vi "onComputeIntervals.vi"(8 "error in (no error)":errorcluster, 9 "Cron Interval":T1, 10 "Expression":string, 11 "Cron.Quartz in":refnum<class "Cron.Quartz.lvclass">) -> (0 "error out":errorcluster, 2 "Interval Parameters":T2, 3 "Cron.Quartz out":refnum<class "Cron.Quartz.lvclass">)   [LabVIEW 2013, in "openCron.lvlib" / "Cron.Quartz.lvclass"]
uses:
  Cron.Quartz.lvclass
  Cron/Cron Interval -- cluster.ctl
  Cron/Cron Interval -- enum.ctl
  Cron/Cron.lvclass
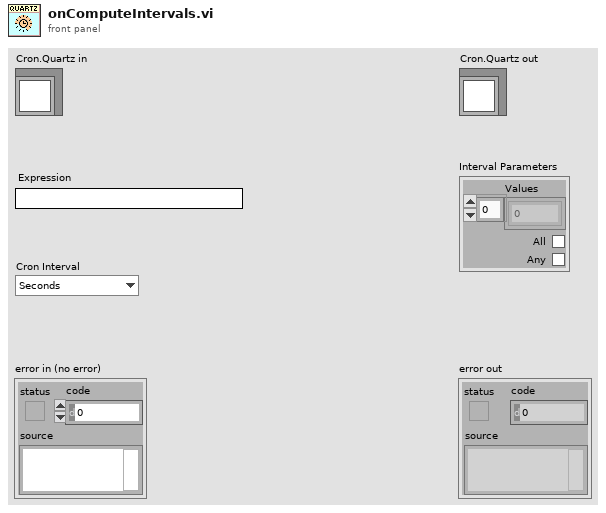
[diagram p1: front panel]
types:
  T1 = typedef "openCron.lvlib/Cron.lvclass/Cron Interval -- enum.ctl" = enum16{"Seconds", "Minutes", "Hours", "Day of Month", "Month", "Day of Week", "Year"}
  T2 = typedef "openCron.lvlib/Cron.lvclass/Cron Interval -- cluster.ctl" = cluster{"Values":i32[], "All":bool, "Any":bool}
  T3 = enum16{"SUN", "MON", "TUE", "WED", "THU", "FRI", "SAT"}
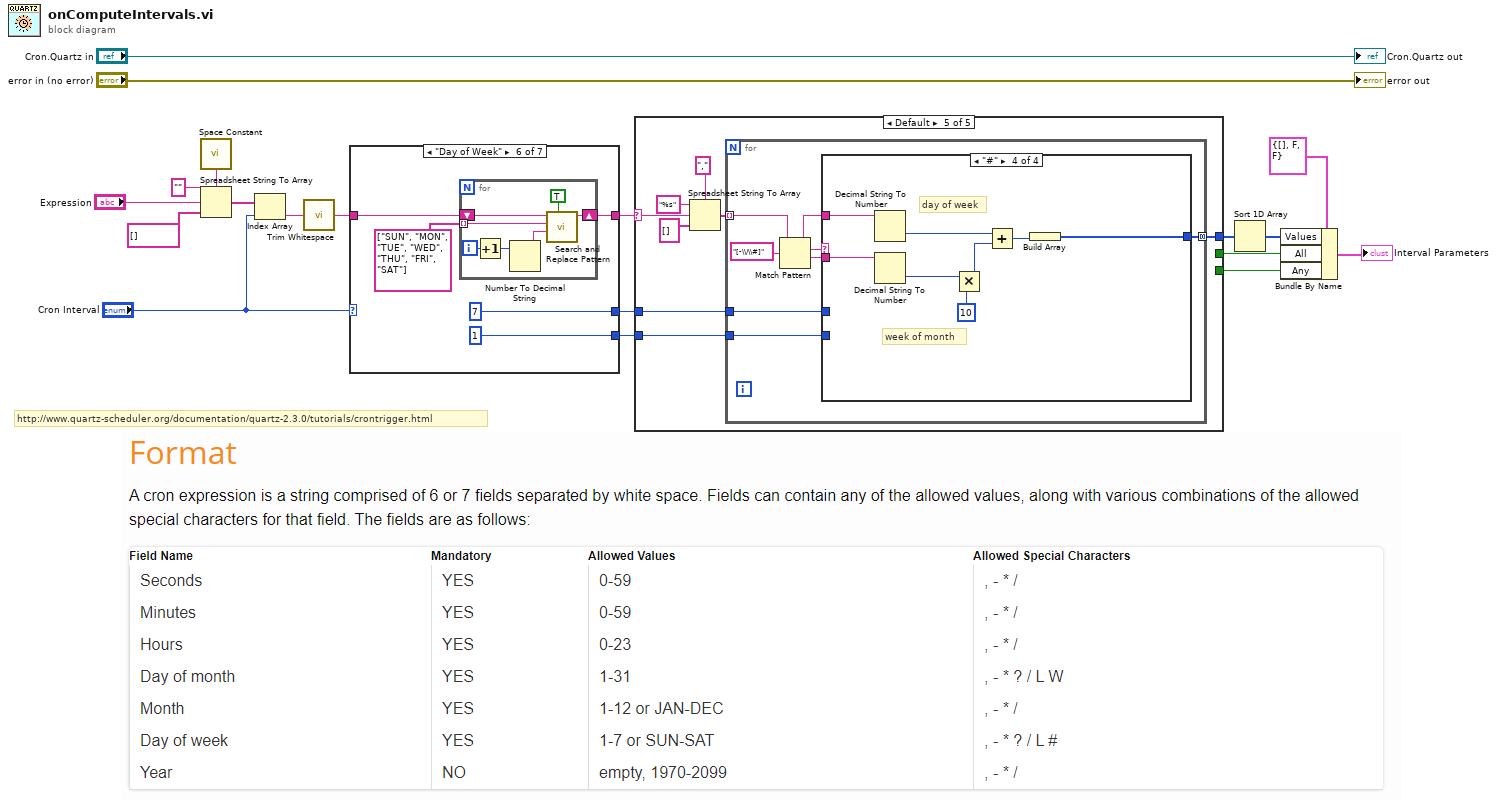
[diagram p0: block diagram]
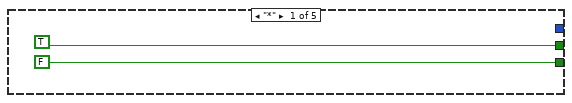
[diagram p2: hidden frame]
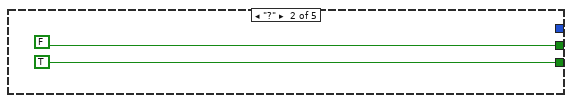
[diagram p3: hidden frame]
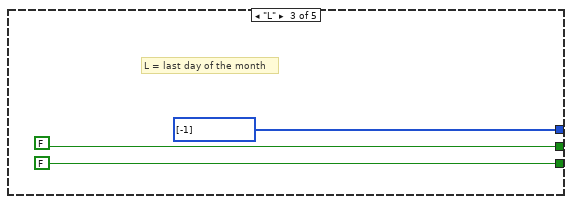
[diagram p4: hidden frame]
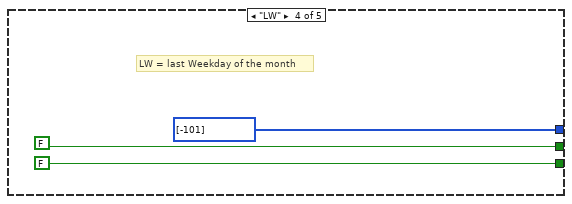
[diagram p5: hidden frame]
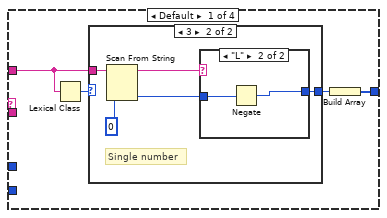
[diagram p6: hidden frame]
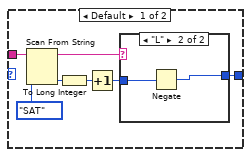
[diagram p7: hidden frame]
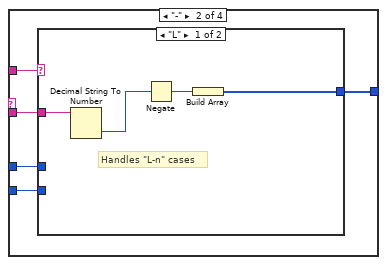
[diagram p10: hidden frame]
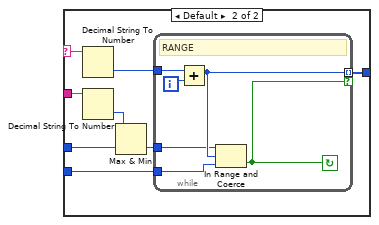
[diagram p11: hidden frame]
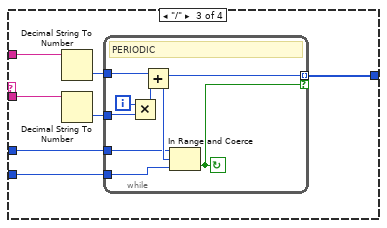
[diagram p12: hidden frame]
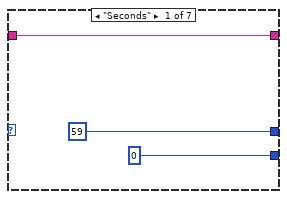
[diagram p13: hidden frame]
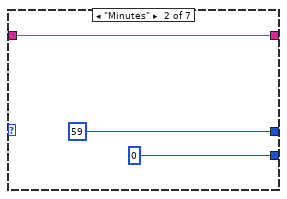
[diagram p14: hidden frame]
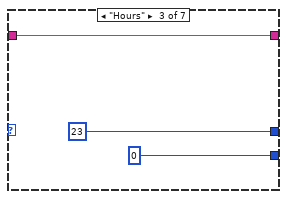
[diagram p15: hidden frame]
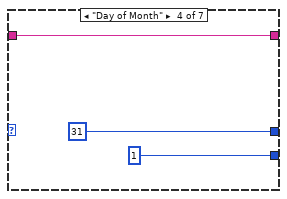
[diagram p16: hidden frame]
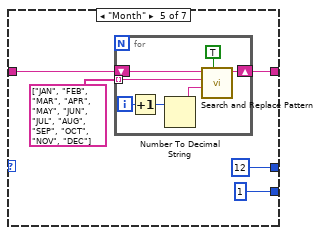
[diagram p17: hidden frame]
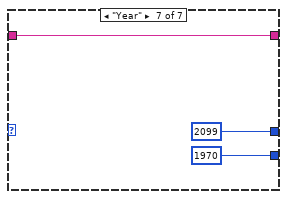
[diagram p18: hidden frame]
diagram:
  # "http://www.quartz-scheduler.org/documentation/quartz-2.3.0/tutorials/crontrigger.html"
  n1 = call <vilib>:"Space Constant.vi"() -> ("String"=w14:string)
  n2 = Spreadsheet String To Array(delimiter (Tab)=w14, format string="", spreadsheet string="Expression", array type (2D Dbl)=string[] []) -> (array=w13:string[])
  n3 = Index Array(array=w13, index="Cron Interval") -> (element=w11:string)
  n4 = call <vilib>:"Trim Whitespace.vi"("string"=w11) -> ("trimmed string"=w2:string)  [unwired: 1 in]
  n5 = case shown="\"Day of Week\"" "Cron Interval" {
    tunnel: [59 ("y") 59 ("y") 23 ("y") 31 ("y") 12 ("y") 7 ("y") 2099 ("y")] -> w10
    tunnel: [0 ("y") 0 ("y") 0 ("y") 1 ("y") 1 ("y") 1 ("y") 1970 ("y")] -> w9
    tunnel: w2 -> [w20 w23 w26 w29 w33 w45 w56]
    tunnel: [w20 w23 w26 w29 w34 w44 w56] -> w1
    frame "Seconds" {
    }
    frame "Minutes" {
    }
    frame "Hours" {
    }
    frame "Day of Month" {
    }
    frame "Month" {
      n6 = for {
        shift-right: [w43] -> w34
        shift-left: w33 -> [w42]
        tunnel: string[] ["JAN", "FEB", "MAR", "APR", "MAY", "JUN", "JUL", "AUG", "SEP", "OCT", "NOV", "DEC"] -> [w40] mode=indexing
        i -> [w39]
        n7 = Increment(x=w39) -> (x+1=w38:i32)
        n8 = Number To Decimal String(number=w38) -> (decimal integer string=w37:string)  [unwired: 1 in]
        n9 = call <vilib>:"Search and Replace Pattern.vi"("string"=w42, "regular expression (\"\")"=w40, "replace string (\"\")"=w37, "replace all? (F)"=TRUE) -> ("result string"=w43:string)  [unwired: 1 in, 1 out]
      }
    }
    frame "Day of Week" {
      n10 = for {
        shift-right: [w55] -> w44
        shift-left: w45 -> [w54]
        tunnel: string[] ["SUN", "MON", "TUE", "WED", "THU", "FRI", "SAT"] -> [w52] mode=indexing
        i -> [w51]
        n11 = Increment(x=w51) -> (x+1=w50:i32)
        n12 = Number To Decimal String(number=w50) -> (decimal integer string=w49:string)  [unwired: 1 in]
        n13 = call <vilib>:"Search and Replace Pattern.vi"("string"=w54, "regular expression (\"\")"=w52, "replace string (\"\")"=w49, "replace all? (F)"=TRUE) -> ("result string"=w55:string)  [unwired: 1 in, 1 out]
      }
    }
    frame "Year" {
    }
  }
  n14 = case shown="Default" w1 {
    selector: w1 -> [_ _ _ _ w72]
    tunnel: [_ _ i32[] [-1] i32[] [-101] w71] -> w7
    tunnel: [TRUE FALSE FALSE FALSE _] -> w6
    tunnel: [FALSE TRUE FALSE FALSE _] -> w5
    tunnel: w10 -> [_ _ _ _ w70]
    tunnel: w9 -> [_ _ _ _ w69]
    frame "*" {
    }
    frame "?" {
    }
    frame "L" {
      # "L = last day of the month"
    }
    frame "LW" {
      # "LW = last Weekday of the month"
    }
    frame Default {
      n15 = Spreadsheet String To Array(delimiter (Tab)=",", format string="%s", spreadsheet string=w72, array type (2D Dbl)=string[] []) -> (array=w73:string[])
      n16 = for {
        tunnel: w73 -> [w84] mode=indexing
        tunnel: [w80] -> w71 mode=concatenating
        tunnel: w70 -> [w78]
        tunnel: w69 -> [w77]
        n17 = Match Pattern(string=w84, regular expression="[-\\/\\#]") -> (before substring=w81:string, match substring=w82:string, after substring=w79:string)  [unwired: 1 in, 1 out]
        n18 = case shown="\"#\"" w82 {
          tunnel: w81 -> [w86 w107 w136 w152]
          tunnel: [w87 w110 w134 w150] -> w80
          tunnel: w79 -> [_ w111 w132 w151]
          tunnel: w78 -> [_ w109 w131 _]
          tunnel: w77 -> [_ w108 w130 _]
          frame Default {
            n19 = Lexical Class(1:w86) -> (0:w85:i16)
            n20 = case shown="3" w85 {
              tunnel: [w89 w101] -> w88
              tunnel: w86 -> [w95 w103]
              frame Default {
                n21 = Scan From String(input string=w95, default 1=T3."SAT" ("y")) -> (remaining string=w91:string, output 1=w92:T3)  [unwired: 3 in, 2 out]
                n22 = To Long Integer(number=w92) -> (32bit integer=w93:i32)
                n23 = Increment(x=w93) -> (x+1=w90:i32)
                n24 = case shown="\"L\"" w91 {
                  tunnel: w90 -> [w96 w98]
                  tunnel: [w96 w97] -> w89
                  frame Default {
                  }
                  frame "L" {
                    n25 = Negate(x=w98) -> (-x=w97:i32)
                  }
                }
              }
              frame 3 {
                # "Single number"
                n26 = Scan From String(input string=w103, default 1=0 ("32bit integer")) -> (remaining string=w102:string, output 1=w99:i32)  [unwired: 3 in, 2 out]
                n27 = case shown="\"L\"" w102 {
                  tunnel: w99 -> [w104 w106]
                  tunnel: [w104 w105] -> w101
                  frame Default {
                  }
                  frame "L" {
                    n28 = Negate(x=w106) -> (-x=w105:i32)
                  }
                }
              }
            }
            n29 = Build Array(w88) -> (w87:i32[])
          }
          frame "-" {
            n30 = case shown="\"L\"" w107 {
              selector: w107 -> [_ w116]
              tunnel: w111 -> [w115 w122]
              tunnel: [w113 w121] -> w110
              tunnel: w109 -> [_ w119]
              tunnel: w108 -> [_ w118]
              frame "L" {
                # "Handles \"L-n\" cases"
                n31 = Decimal String To Number(string=w115) -> (number=w114:i32)  [unwired: 2 in, 1 out]
                n32 = Negate(x=w114) -> (-x=w112:i32)
                n33 = Build Array(w112) -> (w113:i32[])
              }
              frame Default {
                n34 = Decimal String To Number(string=w116) -> (number=w123:i32)  [unwired: 2 in, 1 out]
                n35 = Decimal String To Number(string=w122) -> (number=w120:i32)  [unwired: 2 in, 1 out]
                n36 = Max & Min(x=w120, y=w119) -> (min(x,y)=w117:i32)  [unwired: 1 out]
                n37 = while {
                  tunnel: w123 -> [w129]
                  tunnel: [w126] -> w121 mode=indexing if=w127
                  tunnel: w118 -> [w125]
                  tunnel: w117 -> [w124]
                  i -> [w128]
                  stop <- w127 continue-if-true
                  # "RANGE"
                  n38 = Add(x=w129, y=w128) -> (x+y=w126:i32)
                  n39 = In Range and Coerce(upper limit=w124, x=w126, lower limit=w125) -> (In Range?=w127:bool)  [unwired: 1 out]
                }
              }
            }
          }
          frame "/" {
            n40 = Decimal String To Number(string=w136) -> (number=w135:i32)  [unwired: 2 in, 1 out]
            n41 = Decimal String To Number(string=w132) -> (number=w133:i32)  [unwired: 2 in, 1 out]
            n42 = while {
              tunnel: w135 -> [w144]
              tunnel: [w140] -> w134 mode=indexing if=w137
              tunnel: w133 -> [w143]
              tunnel: w131 -> [w139]
              tunnel: w130 -> [w138]
              i -> [w142]
              stop <- w137 continue-if-true
              # "PERIODIC"
              n43 = Multiply(x=w142, y=w143) -> (x*y=w141:i32)
              n44 = Add(x=w144, y=w141) -> (x+y=w140:i32)
              n45 = In Range and Coerce(upper limit=w139, x=w140, lower limit=w138) -> (In Range?=w137:bool)  [unwired: 1 out]
            }
          }
          frame "#" {
            # "week of month"
            # "day of week"
            n46 = Decimal String To Number(string=w152) -> (number=w147:i32)  [unwired: 2 in, 1 out]
            n47 = Decimal String To Number(string=w151) -> (number=w149:i32)  [unwired: 2 in, 1 out]
            n48 = Multiply(x=w149, y=10) -> (x*y=w146:i32)
            n49 = Add(x=w147, y=w146) -> (x+y=w145:i32)
            n50 = Build Array(w145) -> (w150:i32[])
          }
        }
      }
    }
  }
  n51 = Sort 1D Array(array=w7) -> (sorted array=w8:i32[])
  n52 = Bundle By Name(cluster=T2 {"Values"=[], "All"=FALSE, "Any"=FALSE} ("Interval"), "Values"=w8, "All"=w6, "Any"=w5) -> (→"Interval Parameters":T2)
  "error out" <- "error in (no error)"
  "Cron.Quartz out" <- "Cron.Quartz in"
